vi "tp_essai_1.vi"(8 "error in (no error)":errorcluster, 10 "ID Query (True)":bool=TRUE, 11 "VISA resource name":refnum<visa-resource-name>) -> (0 "error out":errorcluster, 3 "VISA resource name out":refnum<visa-resource-name>)   [LabVIEW 2012]
doc: "Establishes communication with the instrument and optionally performs an instrument identification query and/or an instrument reset. It also places the instrument in a default state needed for other instrument driver operations. Therefore, call this VI before calling other instrument driver VIs for this instrument. Generally, you need to call the <B>Initialize VI</B> only once at the beginning of an application."
uses:
  <instrlib>/Agilent 34401/Agilent 34401.lvlib
panel:
  out "x = y?":bool
  # "(c) 2005-2008 National Instruments.  ALL RIGHTS RESERVED."
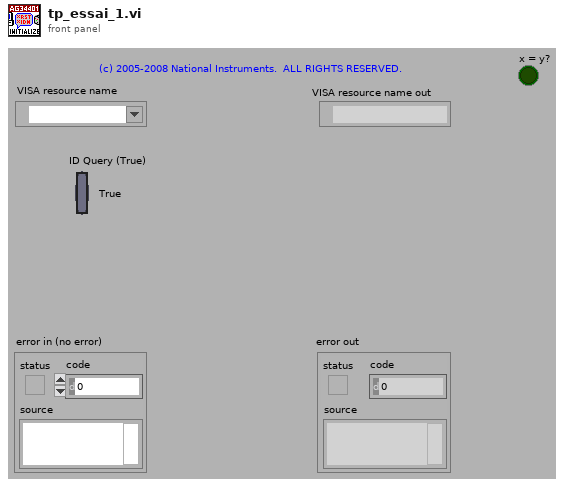
[diagram p1: front panel]
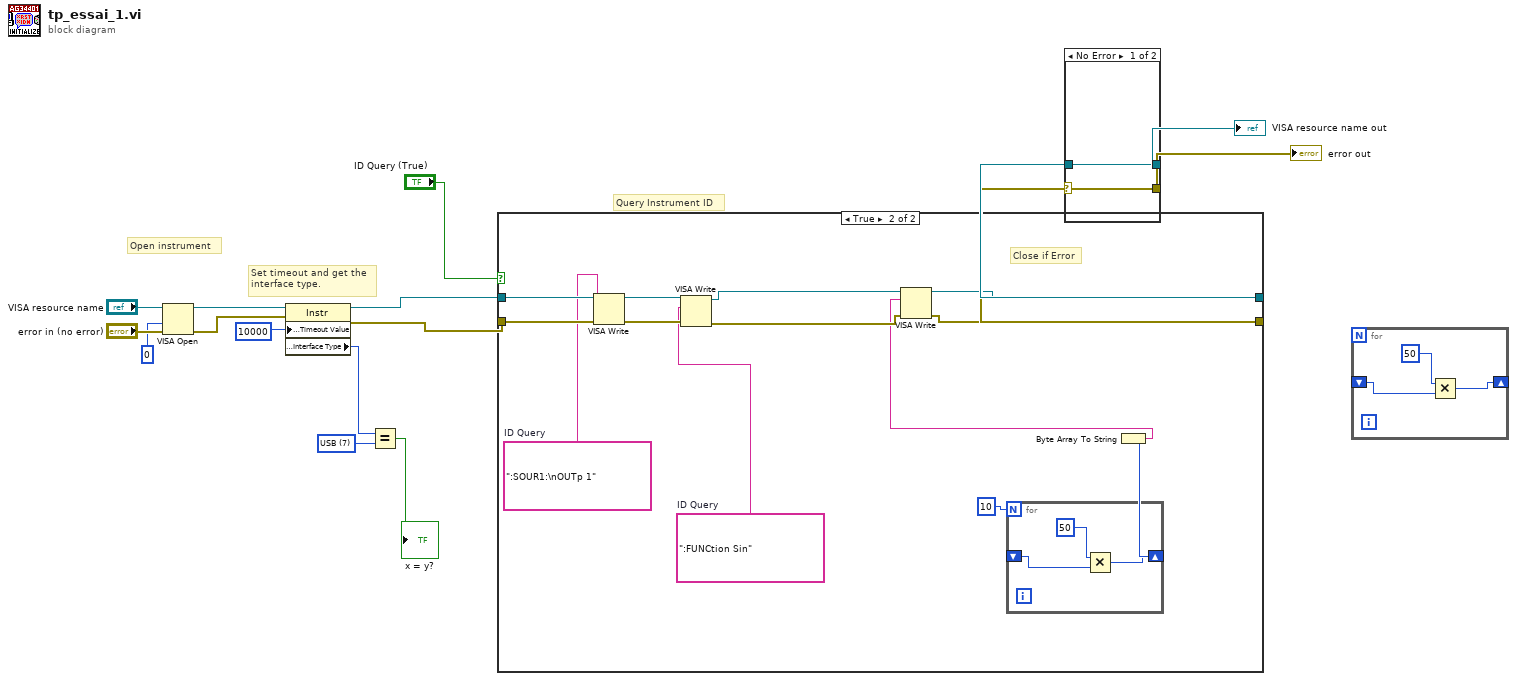
[diagram p0: block diagram]
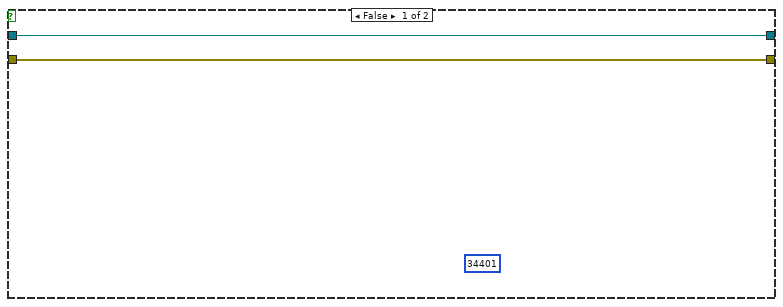
[diagram p2: hidden frame]
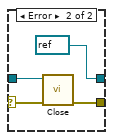
[diagram p3: hidden frame]
diagram:
  w12 = u16 7 items=["GPIB"=1, "VXI"=2, "GPIB-VXI"=3, "Serial"=4, "PXI"=5, "TCPIP"=6, "USB"=7] ("Interface Information:Interface Type")
  # "Set timeout and get the\ninterface type."
  # "Close if Error"
  # "Query Instrument ID"
  # "Open instrument"
  n1 = VISA Open(access mode=u32 0, error in (no error)="error in (no error)", VISA resource name="VISA resource name") -> (VISA resource name=w7:refnum<visa-resource-name>, error out=w6:errorcluster)  [unwired: 2 in]
  n2 = property on="Property Node" class="Instr"(reference=w7, error in=w6, "General Settings:Timeout Value"=u32 10000) -> (reference out=w5:refnum<visa-resource-name>, error out=w4:errorcluster, "Interface Information:Interface Type"=w14:u16)
  n3 = Equal?(x=w14, y=w12) -> (x = y?=→"x = y?":bool)
  n4 = case shown="True" "ID Query (True)" {
    tunnel: [w17 w23] -> w2
    tunnel: [w18 w22] -> w3
    tunnel: w5 -> [w18 w30]
    tunnel: w4 -> [w17 w31]
    frame False {
      (unwired) 34401
    }
    frame True {
      w26 = ":FUNCtion Sin"  # ID Query
      w29 = ":SOUR1:\nOUTp 1"  # ID Query
      n5 = VISA Write(VISA resource name=w30, write buffer=w29, error in (no error)=w31) -> (VISA resource name out=w28:refnum<visa-resource-name>, error out=w27:errorcluster)  [unwired: 1 out]
      n6 = VISA Write(VISA resource name=w28, write buffer=w26, error in (no error)=w27) -> (VISA resource name out=w25:refnum<visa-resource-name>, error out=w24:errorcluster)  [unwired: 1 out]
      n7 = for {
        N: 10 -> [_]
        shift-right: [w32] -> w19
        shift-left: _ -> [w33]
        n8 = Multiply(x=50, y=w33) -> (x*y=w32:i32)
      }
      n9 = Byte Array To String(unsigned byte array=w19) -> (string=w20:string)
      n10 = VISA Write(VISA resource name=w25, write buffer=w20, error in (no error)=w24) -> (VISA resource name out=w22:refnum<visa-resource-name>, error out=w23:errorcluster)  [unwired: 1 out]
    }
  }
  n11 = case shown="No Error" w2 {
    selector: w2 -> [w35 w38]
    tunnel: w3 -> [w36 w39]
    tunnel: [w36 refnum<visa-resource-name> refnum ("VISA resource name out")] -> w10
    tunnel: [w35 w40] -> w8
    frame No Error {
    }
    frame Error {
      n12 = call <instrlib>:"Close.vi"("error in (no error)"=w38, "VISA resource name"=w39) -> ("error out"=w40:errorcluster)  [unwired: 9 in]
    }
  }
  "VISA resource name out" <- w10
  "error out" <- w8
  n13 = for {
    shift-right: [w41] -> _
    shift-left: _ -> [w42]
    n14 = Multiply(x=50, y=w42) -> (x*y=w41:i32)
  }
